vi "IMU Get Euler Angle.vi"   [LabVIEW 2023, in "MrcLib.lvlib"]
doc: "Returns the computed Euler angles of the built-in sensor. Be sure to select the version that matches the orientation of the robot Controller."
uses:
  <vilib>/MRC/MrcLib.lvlib
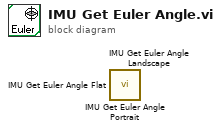
[diagram p0: block diagram]
diagram:
  n1 = call <vilib>:"IMU Get Euler Angle Portrait.vi"() -> ()  [unwired: 9 in, 3 out]
  n2 = call <vilib>:"IMU Get Euler Angle Landscape.vi"() -> ()  [unwired: 9 in, 3 out]
  n3 = call <vilib>:"IMU Get Euler Angle Flat.vi"() -> ()  [unwired: 9 in, 3 out]
